vi "Modif Alarme reg  pour test.vi"() -> ()   [LabVIEW 2022 SP3]
uses:
  Enum/Enum r17.ctl
  Enum/Enum s1.ctl
  Variables globales/Variables glob EUROTHERM.vi
panel:
  in  "par reg":T1(array[cluster])
  in  "sortir":bool
  in  "envoi":bool
  # "Modification des alarmes régulateur pour enclencher les sécurités"
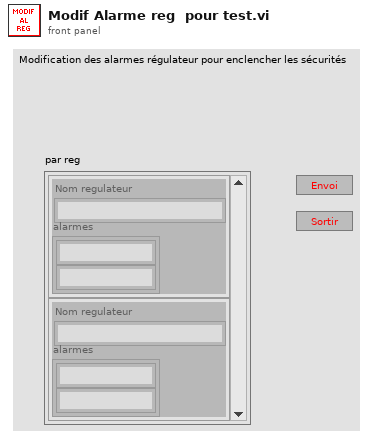
[diagram p1: front panel]
types:
  T1 = cluster{"Nom regulateur":string, "alarmes":string[]}[]
  T2 = typedef "Enum r17.ctl" = enum16{"init", "choix", "envoi", "message", "sortir"}
  T3 = enum8{"Enabled", "Disabled", "Disabled and Grayed Out"}
  T4 = typedef "Enum s1.ctl" = enum16{"Alerte vide", "Alerte temperature min-max", "Alerte temperature ecart", "Alerte Keller", "Alerte compteur", "Alerte régulateurs"}
  T5 = cluster{"Noms voies select acqui 1COM":string[]}[]
  T6 = cluster{"Nom regulateur":string, "alarmes":string[]}
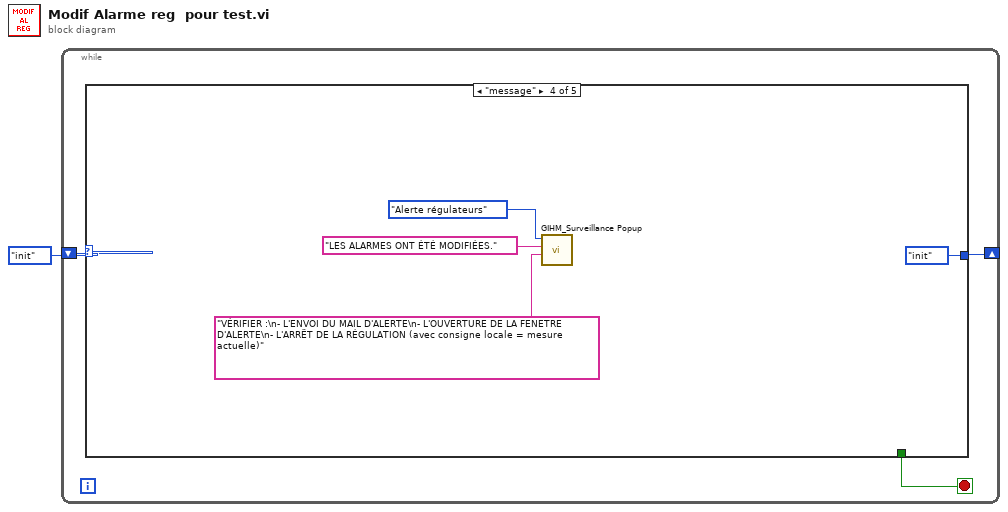
[diagram p0: block diagram]
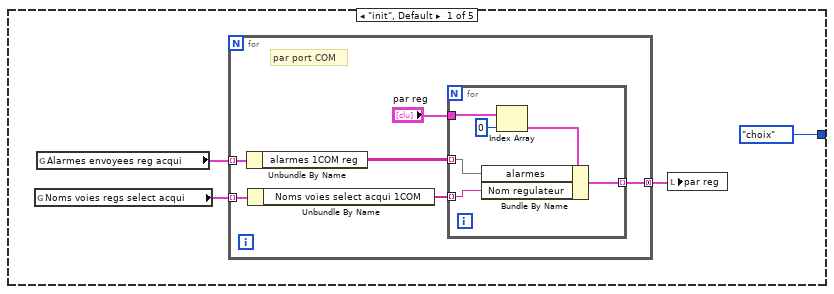
[diagram p2: hidden frame]
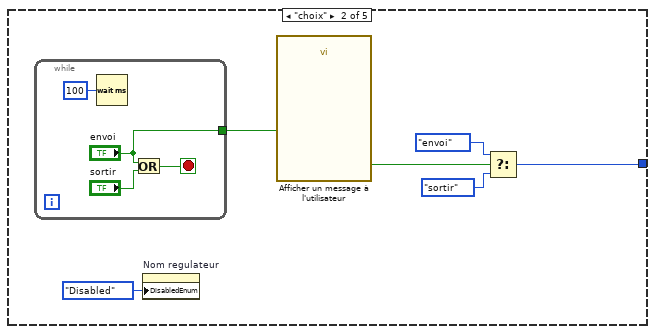
[diagram p3: hidden frame]
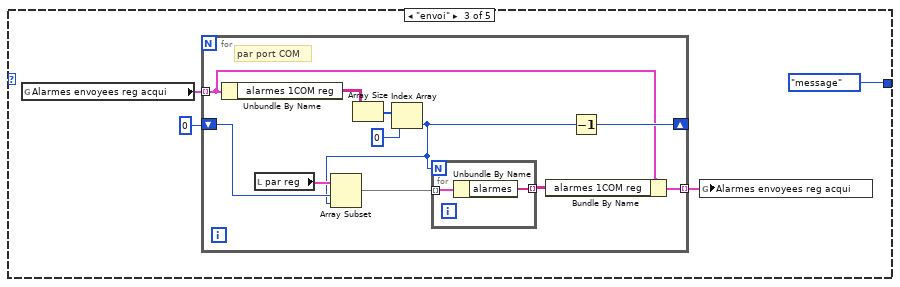
[diagram p4: hidden frame]
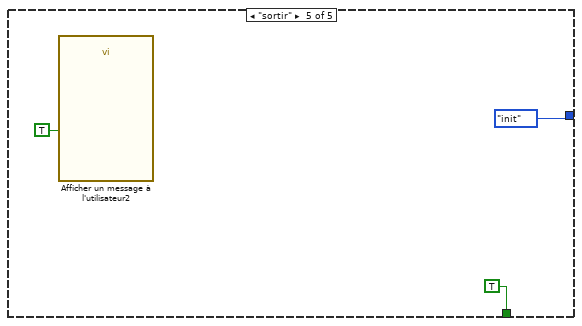
[diagram p5: hidden frame]
diagram:
  n1 = while {
    shift-right: [w3] -> _
    shift-left: Enum_r17."init" ("Énum") -> [w4]
    stop <- w2 stop-if-true
    n2 = case shown="\"message\"" w4 {
      tunnel: [Enum_r17."choix" ("Énum") w24 Enum_r17."message" ("Énum") Enum_r17."init" ("Énum") Enum_r17."init" ("Énum")] -> w3
      tunnel: [_ _ _ _ TRUE] -> w2
      frame "init", Default {
        n3 = global read "Variables glob EUROTHERM.vi" "Noms voies regs select acqui"() -> (w7:T5)
        n4 = global read "Variables glob EUROTHERM.vi" "Alarmes envoyees reg acqui"() -> (w6:cluster{"alarmes 1COM reg":string[][]}[])
        n5 = for {
          tunnel: w6 -> [w14] mode=indexing
          tunnel: w7 -> [w13] mode=indexing
          tunnel: [w9] -> w8 mode=concatenating
          # "par port COM"
          n6 = Unbundle By Name(w14) -> ("alarmes 1COM reg"=w12:string[][])
          n7 = Unbundle By Name(w13) -> ("Noms voies select acqui 1COM"=w11:string[])
          n8 = for {
            tunnel: w12 -> [w17] mode=indexing
            tunnel: w11 -> [w16] mode=indexing
            tunnel: "par reg" -> [w20]
            tunnel: [w15] -> w9 mode=indexing
            n9 = Index Array(array=w20, index=0 ("indice")) -> (element=w18:T6)
            n10 = Bundle By Name(cluster=w18, "alarmes"=w17, "Nom regulateur"=w16) -> (w15:T6)
          }
        }
        n11 = local write "par reg"(w8) -> ()
      }
      frame "choix" {
        n12 = while {
          tunnel: ["envoi"] -> w22
          stop <- w29 stop-if-true
          n13 = Wait (ms)(milliseconds to wait=u32 100 ("attente (ms)")) -> ()  [unwired: 1 out]
          n14 = Or(x="envoi", y="sortir") -> (x .or. y?=w29:bool)
        }
        n15 = property on="Nom regulateur" class="Ch"("DisabledEnum"=T3."Disabled" ("Désactivé")) -> ()  [unwired: 2 in, 2 out]
        n16 = call "Afficher un message à l'utilisateur"("Enable"=w22) -> ("OK"=w23:bool)  [unwired: 9 in, 1 out]
        n17 = Select(t=Enum_r17."envoi" ("Énum"), s=w23, f=Enum_r17."sortir" ("Énum")) -> (s? t:f=w24:T2)
      }
      frame "envoi" {
        n18 = global read "Variables glob EUROTHERM.vi" "Alarmes envoyees reg acqui"() -> (w32:cluster{"alarmes 1COM reg":string[][]}[])
        n19 = for {
          tunnel: w32 -> [w39] mode=indexing
          shift-right: [w40] -> _
          shift-left: 0 -> [w36]
          tunnel: [w37] -> w33 mode=indexing
          # "par port COM"
          n20 = Unbundle By Name(w39) -> ("alarmes 1COM reg"=w45:string[][])
          n21 = local read "par reg"() -> (w42:T1)
          n22 = Array Size(array=w45) -> (size(s)=w44:i32[])
          n23 = Index Array(array=w44, index=0 ("indice")) -> (element=w35:i32)
          n24 = Array Subset(array=w42, index=w36, length=w35) -> (w41:T1)
          n25 = for {
            N: w35 -> [_]
            tunnel: w41 -> [w47] mode=indexing
            tunnel: [w46] -> w38 mode=indexing
            n26 = Unbundle By Name(w47) -> ("alarmes"=w46:string[])
          }
          n27 = Bundle By Name(cluster=w39, "alarmes 1COM reg"=w38) -> (w37:cluster{"alarmes 1COM reg":string[][]})
          n28 = Decrement(x=w35) -> (x-1=w40:i32)
        }
        n29 = global write "Variables glob EUROTHERM.vi" "Alarmes envoyees reg acqui"(w33) -> ()
      }
      frame "message" {
        n30 = call "GIHM_Surveillance Popup.vi"("Message"="VÉRIFIER :\n- L'ENVOI DU MAIL D'ALERTE\n- L'OUVERTURE DE LA FENETRE D'ALERTE\n- L'ARRËT DE LA RÉGULATION (avec consigne locale = mesure actuelle)", "Problème observé"="LES ALARMES ONT ÉTÉ MODIFIÉES.", "Type problème"=Enum_s1."Alerte régulateurs") -> ()  [unwired: 2 in, 1 out]
      }
      frame "sortir" {
        n31 = call "Afficher un message à l'utilisateur2"("Enable"=TRUE) -> ()  [unwired: 9 in, 2 out]
      }
    }
  }
